vi "MenuHandler.vi"(5 "tree control":refnum<vi>, 7 "message queue out":T1, 8 "error in":errorcluster, 9 "parameters":variant, 10 "menu string":string, 11 "module editor node in":refnum<class "module editor node.lvclass">) -> (0 "error out":errorcluster, 1 "refresh tree?":bool, 2 "Unhandled":bool, 3 "module editor node out":refnum<class "module editor node.lvclass">)   [LabVIEW 2013, in "PL Framework Configuration Tool.lvlib" / "module editor node.lvclass"]
uses:
  module editor node.lvclass
  <vilib>/NI/AMC/Message Queue.ctl
  <vilib>/NI/AMC/Message.ctl
  <vilib>/NI/Tools/Keyed Array/KeyedArray.ctl
  TBM Configuration Node/TBM Configuration Node.lvclass
  <vilib>/NI/Tools/Keyed Array/Tools_KeyedArray.lvlib
  <vilib>/NI/AMC/AMC.lvlib
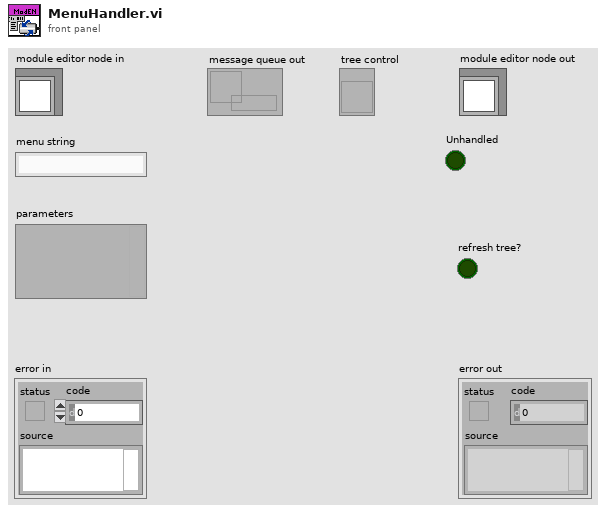
[diagram p1: front panel]
types:
  T1 = typedef "AMC.lvlib/Message Queue.ctl" = refnum<queue>
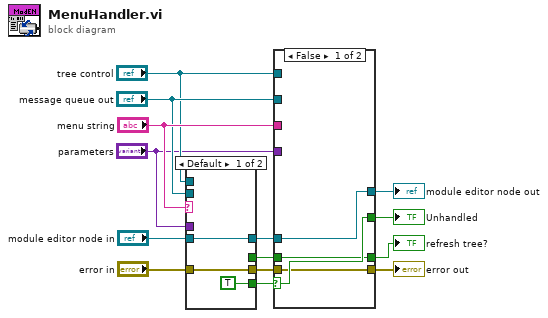
[diagram p0: block diagram]
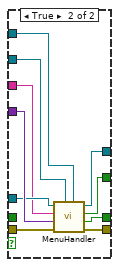
[diagram p2: hidden frame]
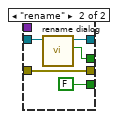
[diagram p3: hidden frame]
diagram:
  n1 = case shown="Default" "menu string" {
    tunnel: [TRUE ("Unhandled") FALSE ("Unhandled")] -> w7
    tunnel: "module editor node in" -> [w16 w20]
    tunnel: [w16 w19] -> w10
    tunnel: [w17 w21] -> w9
    tunnel: "error in" -> [w17 w21]
    tunnel: "message queue out" -> [_ _]
    tunnel: "tree control" -> [_ _]
    tunnel: "parameters" -> [_ _]
    tunnel: [_ w18] -> w1
    frame Default {
    }
    frame "rename" {
      n2 = call "rename dialog.vi"("module editor node in"=w20) -> ("changed"=w18:bool, "module editor node out"=w19:refnum<class "module editor node.lvclass">)  [unwired: 9 in]
    }
  }
  n3 = case shown="False" w7 {
    selector: w7 -> [w26 _]
    tunnel: [w24 w36] -> w14
    tunnel: [w26 w35] -> w13
    tunnel: [w25 w34] -> w12
    tunnel: "tree control" -> [_ w33]
    tunnel: "message queue out" -> [_ w32]
    tunnel: "parameters" -> [_ w31]
    tunnel: w10 -> [w25 w30]
    tunnel: w9 -> [w24 w29]
    tunnel: "menu string" -> [_ w28]
    tunnel: [w23 w27] -> w2
    tunnel: w1 -> [w23 _]
    frame False {
    }
    frame True {
      n4 = call-parent "MenuHandler.vi"("tree control"=w33, "main message queue"=w32, "error in"=w29, "parameters"=w31, "menu string"=w28, "NISE_CEF_serializable node in"=w30) -> ("error out"=w36:errorcluster, "refresh tree?"=w27:bool, "Unhandled"=w35:bool, "NISE_CEF_serializable node out"=w34:refnum<class "module editor node.lvclass">)  [unwired: 2 in]
    }
  }
  "error out" <- w14
  "module editor node out" <- w12
  "Unhandled" <- w13
  "refresh tree?" <- w2
